vi "Advance Market.vi"(8 "error in":errorcluster) -> (0 "error out":errorcluster, 2 "news ticker":string, 3 "price chart":dbl[][](array[numeric]))   [LabVIEW 2020, in "Full Featured MCP Server.lvlib"]
doc: "Advances the simulated market by one second and returns what the front panel shows: the price chart of the last ten minutes (every stock starts at 100) and the news ticker. main.vi calls it once per second."
uses:
  Full Featured MCP Server.lvlib
  Market/Market Mode.ctl
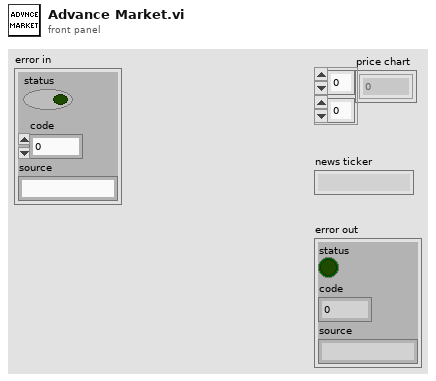
[diagram p1: front panel]
types:
  T1 = typedef "Full Featured MCP Server.lvlib/Market Mode.ctl" = enum16{"Get", "Init", "Advance", "Buy", "Sell"}
  T2 = cluster{"tick":i32, "price history":dbl[][], "shock":dbl[], "momentum":dbl[], "nervousness":dbl[], "mood":dbl, "tension":dbl, "sector mood":dbl[], "news":cluster{"tick":i32, "headline":string, "stocks":i32[], "direction":string}[], "stories":cluster{"arc":i32, "step":i32, "due":i32, "stock":i32, "other":i32}[], "owned":i32[], "wallet":dbl}
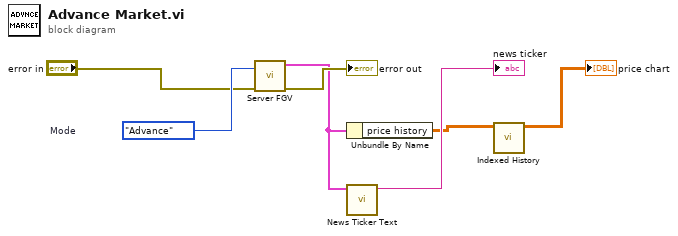
[diagram p0: block diagram]
diagram:
  w2 = Market_Mode."Advance"  # Mode
  n1 = call "Server FGV.vi"("Mode"=w2, "error in"="error in") -> ("error out"=→"error out":errorcluster, "market"=w3:T2)  [unwired: 7 in, 1 out]
  n2 = Unbundle By Name(w3) -> ("price history"=w5:dbl[][])
  n3 = call "News Ticker Text.vi"("market"=w3) -> ("text"=→"news ticker":string)  [unwired: 10 in]
  n4 = call "Indexed History.vi"("price history"=w5) -> ("indexed history"=→"price chart":dbl[][])  [unwired: 10 in]
